vi "Supervisor_Start_Test.vi"(8 "error in (no error)":errorcluster={"status"=FALSE, "code"=0, "source"="\"\""}, 10 "readiness":string, 11 "Approved plan":string) -> (0 "error out":errorcluster={"status"=FALSE, "code"=0, "source"="\"\""}, 2 "status ok":bool, 3 "RunContext/run ID":string)   [LabVIEW 2026]
doc: "INTENT: Establish a new test run. LOGIC: Check interlocks, acquire test ownership token, initialize counters/logging; authorize scheduler."
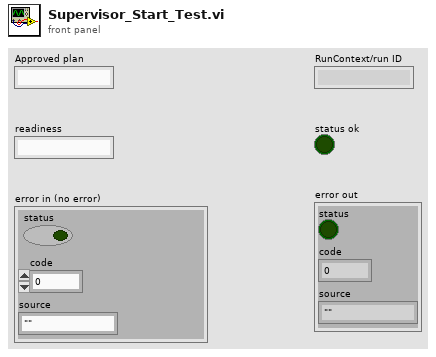
[diagram p1: front panel]
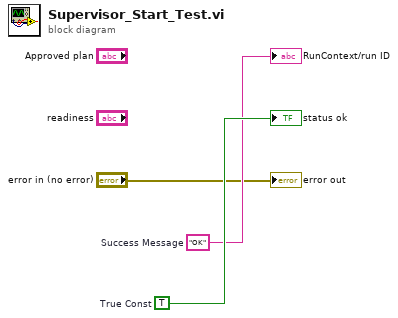
[diagram p0: block diagram]
diagram:
  w3 = TRUE  # True Const
  w2 = "OK"  # Success Message
  "RunContext/run ID" <- w2
  "status ok" <- w3
  "error out" <- "error in (no error)"
